vi "Set Stop Threshold.vi"(7 "nStopThrsh":i32, 8 "error in (no error)":errorcluster caption="错误输入（无错误）", 9 "nChannel":i32, 10 "nBoard":i32, 11 "nDevId":i32) -> (0 "error out":errorcluster caption="错误输出", 3 "function return":i32)   [LabVIEW 2017, in "smncsftmt.lvlib"]
doc: "__declspec(dllexport) int SetStopThreshold(int nDevId, int nBoard, int nChannel, int nStopThrsh);"
uses:
  smncsftmt.lvlib
  smncsftmt.dll
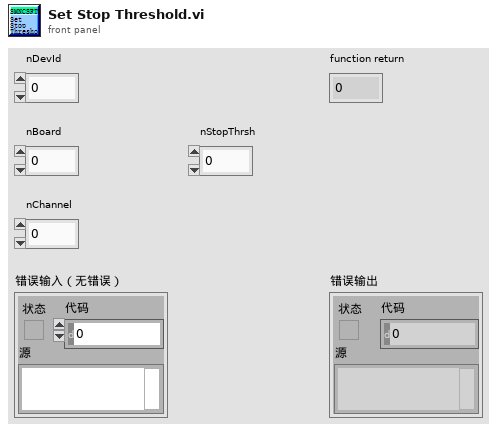
[diagram p1: front panel]
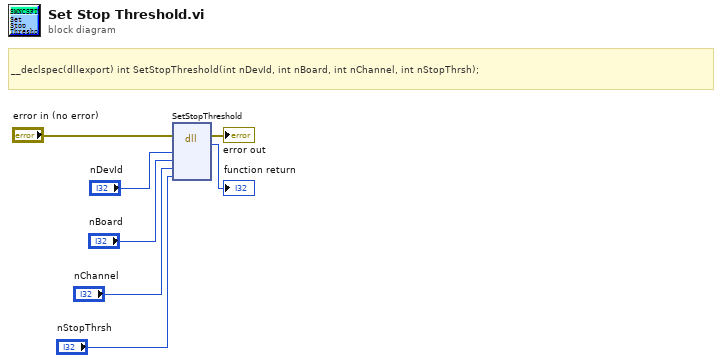
[diagram p0: block diagram]
diagram:
  # "__declspec(dllexport) int SetStopThreshold(int nDevId, int nBoard, int nChannel, int nStopThrsh);"
  n1 = dll-call lib="PTH2oabs CUsersaDesktop\nLABVIEW范例National InstrumentsLabVIEW 2017user.lib\tsmncsftmtsmncsftmt.*" fn="SetStopThreshold"(error in="error in (no error)", "nDevId"="nDevId", "nBoard"="nBoard", "nChannel"="nChannel", "nStopThrsh"="nStopThrsh") -> (error out=→"error out":errorcluster, →"function return":i32)  [unwired: 6 in, 1 out]
